vi "get_item_type.vi"(8 "error in (no error)":errorcluster, 11 "Item in":refnum<class "Item.lvclass">) -> (0 "error out":errorcluster, 2 "item_type":T1, 3 "Item out":refnum<class "Item.lvclass">)   [LabVIEW 2020, in "toml_edit.lvlib" / "Item.lvclass"]
uses:
  Item.lvclass
  type--enum.ctl
  Item.lvclass/Item.ctl
  toml_edit.lvlib
  dragon_toml_64.dll
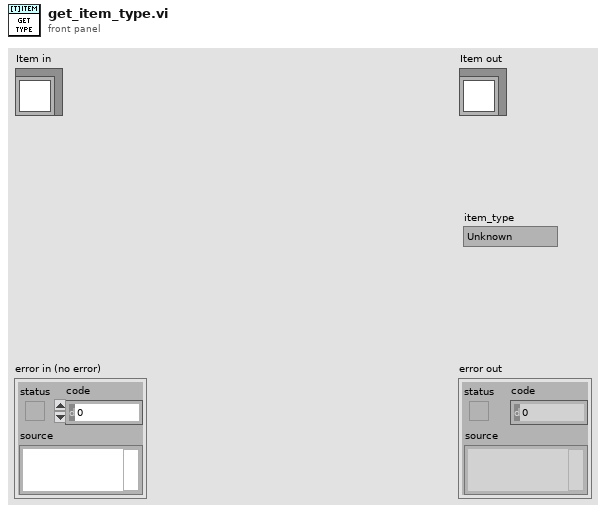
[diagram p1: front panel]
types:
  T1 = typedef "toml_edit.lvlib/Item.lvclass/type--enum.ctl" = enum16{"Unknown", "None", "Value", "ArrayOfTables", "Table"}
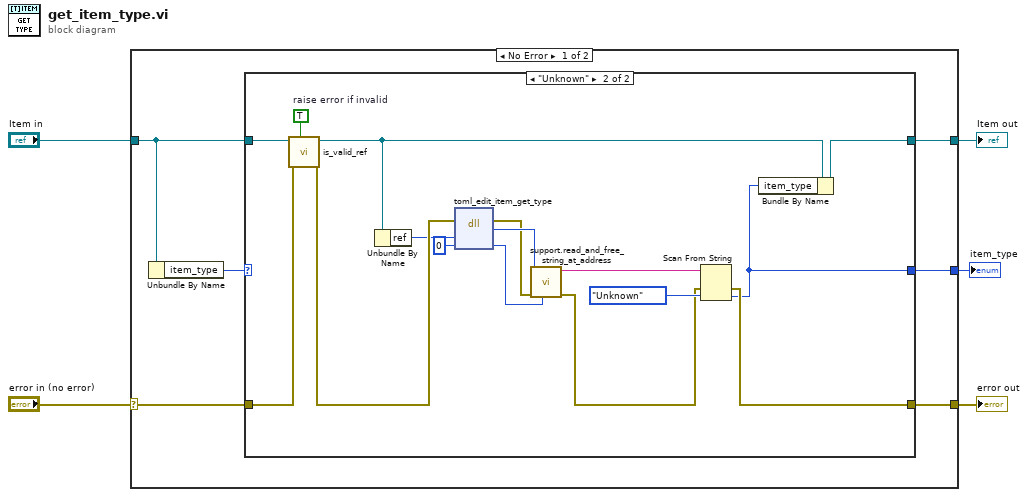
[diagram p0: block diagram]
diagram:
  n1 = case shown="No Error" "error in (no error)" {
    selector: "error in (no error)" -> [w11 w32]
    tunnel: [w10 w32] -> w4
    tunnel: [w9 w31] -> w2
    tunnel: "Item in" -> [w7 w31]
    tunnel: [w8 _] -> w1
    frame No Error {
      n2 = Unbundle By Name(w7) -> ("item_type"=w6:T1)
      n3 = case shown="\"Unknown\"" w6 {
        selector: w6 -> [w13 _]
        tunnel: w11 -> [w12 w24]
        tunnel: [w12 w30] -> w10
        tunnel: [w14 w29] -> w9
        tunnel: [w13 w28] -> w8
        tunnel: w7 -> [w14 w26]
        frame Default {
        }
        frame "Unknown" {
          w17 = TRUE  # raise error if invalid
          n4 = call-dynamic "is_valid_ref.vi"("raise error if invalid? (False)"=w17, "error in (no error)"=w24, "Item in"=w26) -> ("error out"=w25:errorcluster, "Item out"=w27:refnum<class "Item.lvclass">)  [unwired: 6 in, 1 out]
          n5 = Unbundle By Name(w27) -> ("ref"=w21:u64)
          n6 = dll-call lib="C:/projects/dragon-desktop/source/submodules/toml-edit-labview/lv_src/dragon_toml_*.*" fn="toml_edit_item_get_type"(error in=w25, "item_ref"=w21, "string_length"=u32 0) -> (error out=w22:errorcluster, "string_ptr"=w23:u64, "string_length"=w16:u32)  [unwired: 3 in, 1 out]
          n7 = call "support.read_and_free_string_at_address.vi"("string_length"=w16, "error in (no error)"=w22, "string_ptr"=w23) -> ("error out"=w18:errorcluster, "string"=w19:string)  [unwired: 7 in]
          n8 = Scan From String(input string=w19, error in=w18, default 1=type--enum."Unknown" ("type")) -> (error out=w30:errorcluster, output 1=w28:T1)  [unwired: 2 in, 2 out]
          n9 = Bundle By Name(cluster=w27, "item_type"=w28) -> (w29:refnum<class "Item.lvclass">)
        }
      }
    }
    frame Error {
    }
  }
  "error out" <- w4
  "Item out" <- w2
  "item_type" <- w1
